vi "Remplacer_tab.vi"(1 "Nouvel élément/sous tableau":dbl[](array[numeric]), 2 "A partir de":i32, 4 "Tableau":dbl[](array[numeric])) -> (0 "Tableau inséré/remplacé":dbl[](array[numeric]))   [LabVIEW 2022 SP3]
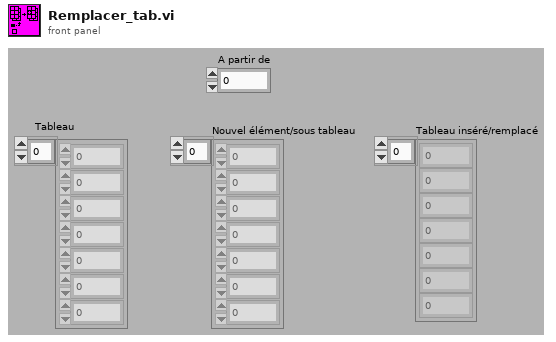
[diagram p1: front panel]
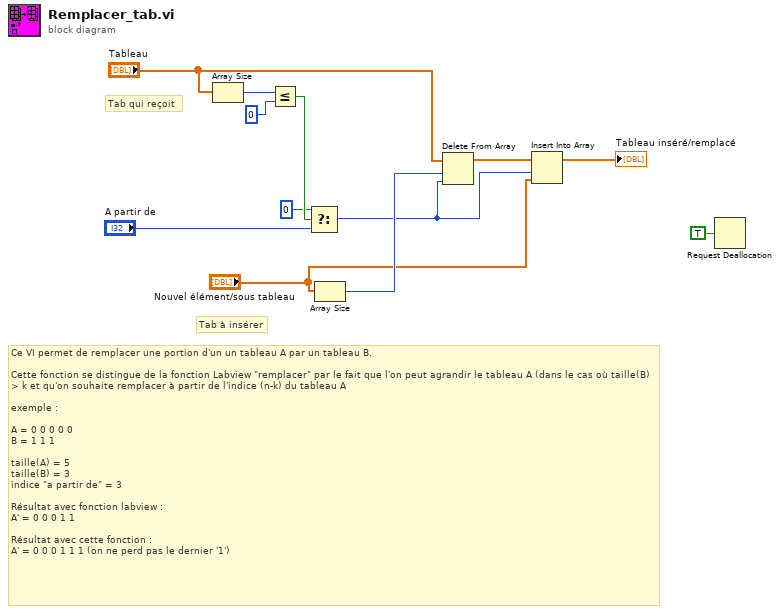
[diagram p0: block diagram]
diagram:
  # "Ce VI permet de remplacer une portion d'un un tableau A par un tableau B. \n\nCette fonction se distingue de la fonction Labview \"remplacer\" par le fait que l'on peut agrandir le tableau A (dans le cas où taille(B) > k et qu'on souhaite remplacer à partir de l'indice (n-k) du tableau A\n\nexemple : \n\nA = 0 0 0 0 0\nB = 1 1 1\n\ntaille(A) = 5\ntaille(B) = 3\nindice \"a partir de\" = 3\n\nRésultat avec fonction labview : \nA' = 0 0 0 1 1\n\nRésultat avec cette fonction :\nA' = 0 0 0 1 1 1 (on ne perd pas le dernier '1')"
  # "Tab à insérer"
  # "Tab qui reçoit"
  n1 = Array Size(array="Tableau") -> (size(s)=w6:i32)
  n2 = Less Or Equal?(x=w6, y=0) -> (x <= y?=w4:bool)
  n3 = Select(t=0 ("cas vrai"), s=w4, f="A partir de") -> (s? t:f=w8:i32)
  n4 = Array Size(array="Nouvel élément/sous tableau") -> (size(s)=w12:i32)
  n5 = Delete From Array(array="Tableau", length=w12, index=w8) -> (array with subset deleted=w11:dbl[])  [unwired: 1 out]
  n6 = Insert Into Array(array=w11, index=w8, new element="Nouvel élément/sous tableau") -> (→"Tableau inséré/remplacé":dbl[])
  n7 = Request Deallocation(TRUE ("flag")) -> ()
